vi "Execute with Process Model Explicit Model.vi"() -> ()   [LabVIEW 2020]
uses:
  SequenceFile/Get Process Model.vi
  SequenceFile/Get Path.vi
  Execution/Set Entry Sequence.vi
  Execution/Set Sequence File.vi
  Execution/Set Process Model.vi
  Execution/Get Result Status.vi
  SequenceFile/SequenceFile.lvclass
  Engine/Engine.lvclass
  Execution/Execution.lvclass
panel:
  in  "Entry Point":string="Single Pass"
  out "Status":string
  in  "Model":T1(tab)
  out "File Model Name":string
  out "Station Model Name":string
  in  "Model Path":path
  in  "SequenceFile Path":path=path "C:/Users/Public/Documents/National Instruments/TestStand 2019 (32-bit)/Examples/Demos/Computer Motherboard Test/LabVIEW/Computer Motherboard Test Sequence.seq"
  # "1."
  # "2."
  # "3."
  # "4."
  # "1. Select the sequence file you'd like to run.\n\n2. Configure the process model you want to run with.\n\n3. If specifying a specific model, select the model file to run with. Otherwise the indicator will update to show the process model that will be used based on the file / station configuration.\n\n4. Enter the name of the entry point to use in the process model. This is usually 'Test UUTs' or 'Single Pass' for models that ship with TestStand."
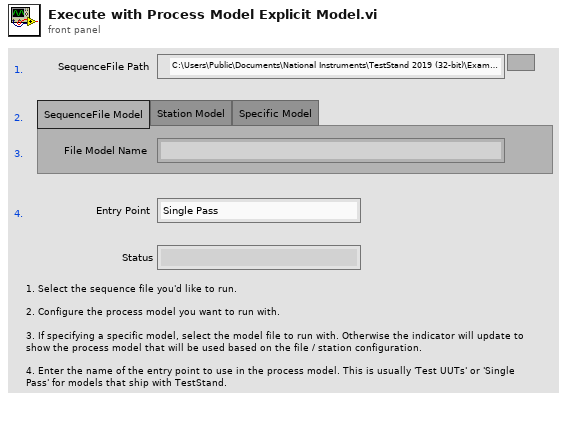
[diagram p1: front panel]
types:
  T1 = enum32{"SequenceFile Model", "Station Model", "Specific Model"}
  T2 = typedef "TSS.lvlib/Engine.lvclass/Session Handle.ctl" = refnum<data-value>
  T3 = typedef "TSS.lvlib/SequenceFile.lvclass/Session Handle.ctl" = refnum<data-value>
  T4 = typedef "TSS.lvlib/Execution.lvclass/Session Handle.ctl" = refnum<data-value>
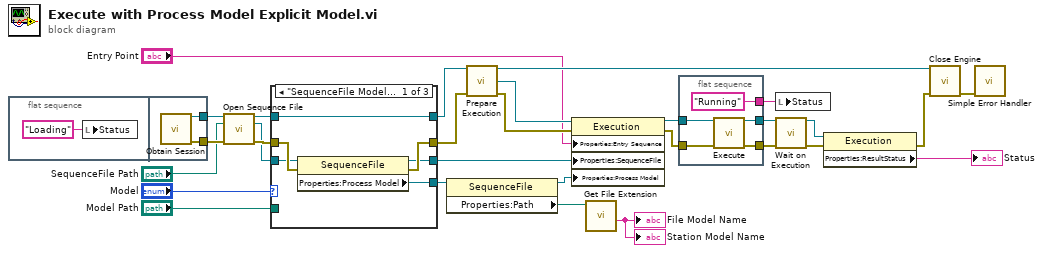
[diagram p0: block diagram]
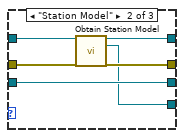
[diagram p2: hidden frame]
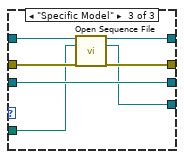
[diagram p3: hidden frame]
diagram:
  n1 = flat-sequence {
    tunnel: [w32] -> w26
    tunnel: [w31] -> w13
    frame #0 {
      n2 = local write "Status"("Loading" ("Status")) -> ()
    }
    frame #1 {
      n3 = call "Obtain Session.vi"() -> ("Session Handle"=w32:T2, "error out"=w31:errorcluster)  [unwired: 14 in]
    }
  }
  n4 = call "Open Sequence File.vi"("Engine in"=w26, "File Path"="SequenceFile Path", "error in (no error)"=w13) -> ("Session Handle out"=w25:T2, "SequenceFile"=w24:T3, "error out"=w29:errorcluster)  [unwired: 10 in]
  n5 = case shown="\"SequenceFile Model\"" "Model" {
    tunnel: "Model Path" -> [_ _ w45]
    tunnel: w25 -> [w33 w44 w50]
    tunnel: w24 -> [w36 w42 w51]
    tunnel: [w35 w39 w46] -> w23
    tunnel: [w33 w43 w49] -> w20
    tunnel: [w34 w42 w51] -> w9
    tunnel: w29 -> [w38 w41 w48]
    tunnel: [w37 w40 w47] -> w12
    frame "SequenceFile Model" {
      n6 = property class="SequenceFile"(reference=w36, error in=w38) -> (reference out=w34:T3, error out=w37:errorcluster, "Properties:Process Model"=w35:T3)
    }
    frame "Station Model" {
      n7 = call "Obtain Station Model.vi"("Session Handle in"=w44, "error in (no error)"=w41) -> ("Session Handle out"=w43:T2, "Station Model"=w39:T3, "error out"=w40:errorcluster)  [unwired: 11 in]
    }
    frame "Specific Model" {
      n8 = call "Open Sequence File.vi"("Engine in"=w50, "File Path"=w45, "error in (no error)"=w48) -> ("Session Handle out"=w49:T2, "SequenceFile"=w46:T3, "error out"=w47:errorcluster)  [unwired: 10 in]
    }
  }
  n9 = property class="SequenceFile"(reference=w23) -> (reference out=w18:T3, "Properties:Path"=w22:path)  [unwired: 1 in, 1 out]
  n10 = call "Prepare Execution.vi"("Session Handle in"=w20, "error in (no error)"=w12) -> ("Session Handle out"=w10:T2, "Execution"=w19:T4, "error out"=w11:errorcluster)  [unwired: 11 in]
  n11 = property class="Execution"(reference=w19, error in=w11, "Properties:Entry Sequence"="Entry Point", "Properties:SequenceFile"=w9, "Properties:Process Model"=w18) -> (reference out=w17:T4, error out=w14:errorcluster)
  n12 = call <vilib>:"Get File Extension.vi"("file"=w22) -> ("filename without extension"=→"File Model Name" →"Station Model Name":string)  [unwired: 6 in, 4 out]
  n13 = flat-sequence {
    tunnel: w17 -> [w56]
    tunnel: [w55] -> w16
    tunnel: [w54] -> w15
    tunnel: w14 -> [w53]
    tunnel: ["Running" ("Status")] -> w3
    frame #0 {
      n14 = call "Execute.vi"("Session Handle in"=w56, "error in (no error)"=w53) -> ("Session Handle out"=w55:T4, "error out"=w54:errorcluster)  [unwired: 12 in]
    }
  }
  n15 = local write "Status"(w3) -> ()
  n16 = call "Wait on Execution.vi"("Session Handle in"=w16, "error in (no error)"=w15) -> ("Session Handle out"=w8:T4, "error out"=w7:errorcluster)  [unwired: 11 in, 1 out]
  n17 = property class="Execution"(reference=w8, error in=w7) -> (error out=w1:errorcluster, "Properties:ResultStatus"=→"Status":string)  [unwired: 1 out]
  n18 = call "Close Engine.vi"("Session Handle in"=w10, "error in (no error)"=w1) -> ("error out"=w5:errorcluster)  [unwired: 13 in]
  n19 = call <vilib>:"Simple Error Handler.vi"("error in (no error)"=w5) -> ()  [unwired: 4 in, 5 out]
